vi "Update Message Converter VIs in Unary Method Call.vi"(6 "RPC Method Parameters":T1, 7 "Library":refnum<vi>, 8 "error in (no error)":errorcluster, 11 "VI in":refnum<vi>) -> (0 "error out":errorcluster, 3 "VI out":refnum<vi>)   [LabVIEW 2019, in "gRPC Template Creation Utility.lvlib"]
uses:
  gRPC Template Creation Utility.lvlib
  TypeDefs/RPC Method Parameters.ctl
  OneOf Constants/OneOfConstantsEnum.ctl
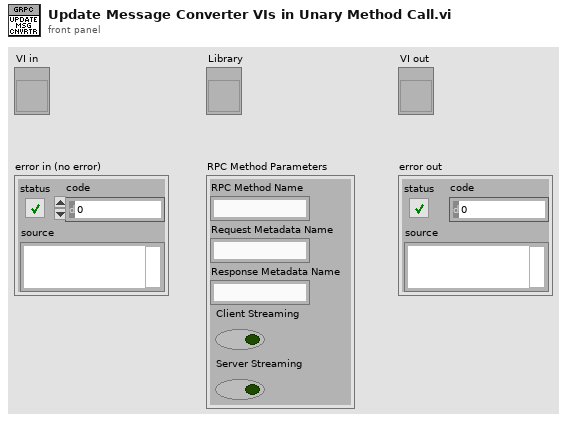
[diagram p1: front panel]
types:
  T1 = typedef "gRPC Template Creation Utility.lvlib/RPC Method Parameters.ctl" = cluster{"RPC Method Name":string, "Request Metadata Name":string, "Response Metadata Name":string, "Client Streaming":bool, "Server Streaming":bool}
  T2 = typedef "gRPC Template Creation Utility.lvlib/OneOfConstantsEnum.ctl" = enum16{"FlatToRichVIPrefix", "RichToFlatVIPrefix", "FlatTypeDefSuffix"}
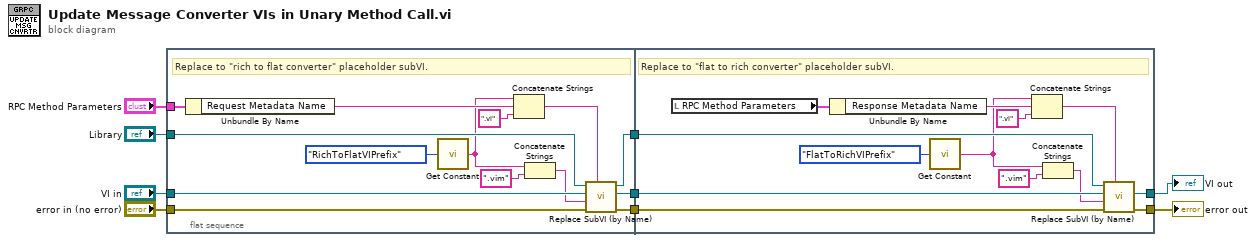
[diagram p0: block diagram]
diagram:
  n1 = flat-sequence {
    tunnel: "RPC Method Parameters" -> [w22]
    tunnel: "error in (no error)" -> [w15]
    tunnel: "Library" -> [w14]
    tunnel: "VI in" -> [w13]
    tunnel: [w18] -> w5
    tunnel: [w17] -> w4
    tunnel: [w16] -> w3
    tunnel: w5 -> [w34]
    tunnel: w4 -> [w35]
    tunnel: w3 -> [w36]
    tunnel: [w33] -> w2
    tunnel: [w32] -> w1
    frame #0 {
      # "Replace to \"rich to flat converter\" placeholder subVI."
      n2 = Unbundle By Name(w22) -> ("Request Metadata Name"=w21:string)
      n3 = call "Get Constant.vi"("Selection"=OneOfConstantsEnum."RichToFlatVIPrefix") -> ("String"=w10:string)
      n4 = Concatenate Strings(w10, w21, ".vi" ("string")) -> (w20:string)
      n5 = Concatenate Strings(w10, ".vim" ("SubVI Name")) -> (w11:string)
      n6 = call "Replace SubVI (by Name).vi"("SubVI to replace with"=w20, "error in (no error)"=w15, "SubVI being replaced"=w11, "VI in"=w13, "Library in"=w14) -> ("error out"=w16:errorcluster, "VI out"=w17:refnum<vi>, "Library out"=w18:refnum<vi>)  [unwired: 4 in]
    }
    frame #1 {
      # "Replace to \"flat to rich converter\" placeholder subVI."
      n7 = local read "RPC Method Parameters"() -> (w30:T1)
      n8 = Unbundle By Name(w30) -> ("Response Metadata Name"=w31:string)
      n9 = call "Get Constant.vi"("Selection"=OneOfConstantsEnum."FlatToRichVIPrefix") -> ("String"=w24:string)
      n10 = Concatenate Strings(w24, w31, ".vi" ("string")) -> (w28:string)
      n11 = Concatenate Strings(w24, ".vim" ("SubVI Name")) -> (w25:string)
      n12 = call "Replace SubVI (by Name).vi"("SubVI to replace with"=w28, "error in (no error)"=w36, "SubVI being replaced"=w25, "VI in"=w35, "Library in"=w34) -> ("error out"=w33:errorcluster, "VI out"=w32:refnum<vi>)  [unwired: 4 in, 1 out]
    }
  }
  "error out" <- w2
  "VI out" <- w1
